vi "Scalar Bitpacked.vi"(8 "error in (no error)":errorcluster, 11 "Node Ptr":T1 format="%.0x") -> (0 "error out":errorcluster)   [LabVIEW 2020, in "FPGA Addon System Explorer.lvlib"]
uses:
  FPGA Addon System Explorer.lvlib
  <vilib>/NI VeriStand/Custom Device API/Custom Device API.lvlib
  Addon Shared/FPGA Addon Shared.lvlib
  Addon Shared/Types/FG Action.ctl
  Addon Shared/SubVIs/Constants.vi
  <vilib>/NI VeriStand/Custom Device API/Get Item Property (String).vi
  <vilib>/NI VeriStand/Custom Device API/Custom Device Item Ref.ctl
panel:
  out "Original Name":string
  in  "SHDocVw.IWebBrowser":refnum<k7>(container)
  in  "Reset":bool
  in  "Apply":bool
  in  "Number of Channels":u8
  in  "Header 2":cluster{"Section Name":string}={"Section Name"="Bitpacked Settings"}
  in  "Header":cluster{"Section Name":string}={"Section Name"="Section Settings"}
  in  "Description":string
  in  "Name":string
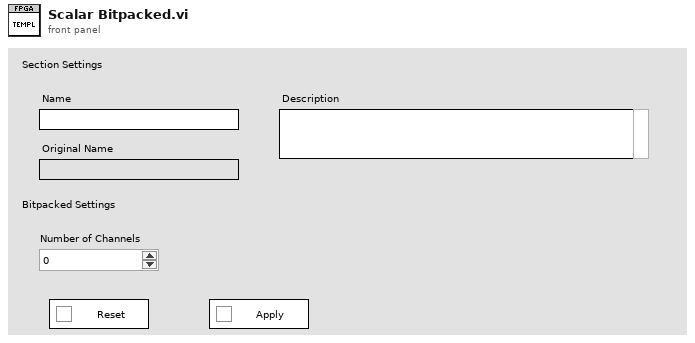
[diagram p1: front panel]
types:
  T1 = typedef "Custom Device API.lvlib/Custom Device Item Ref.ctl" = u64
  T2 = typedef "FPGA Addon Shared.lvlib/FG Action.ctl" = enum8{"GET", "SET"}
  T3 = typedef "FPGA Addon Shared.lvlib/Scalar Settings.ctl" = cluster{"Number of Channels":u8}
  T4 = typedef "FPGA Addon Shared.lvlib/Register Information.ctl" = cluster{"Name":string, "Data Type":T5, "Default Value":variant, "Attributes":variant}
  T5 = typedef "FPGA Addon Shared.lvlib/FPGA Addon Data Type.ctl" = enum8{"<Null>", "I8", "I16", "I32", "I64", "U8", "U16", "U32", "U64", "SGL", "Boolean", "Analog PWM In Settings", "Analog PWM In", "Digital PWM In Settings", "Digital PWM In", "Digital PWM Out", "Sine Out", "FXP", "FXP+/-24.5", "FXP+/-16.5", "FXP+/-32.8", "FXP+/-64.32", "FXP+/-16.7", "FXP+/-20.5", "FXP+/-27.5", "FXP+/-32.16", "FXP+16.3", "FXP+18.3", "Digital Static In", "Digital Static Out", "Digital Static In Settings", "Digital WSS Out", "Quad Encoder Settings", "Quad Encoder In", "Group"}
  T6 = typedef "Custom Device API.lvlib/Custom Device Item Info.ctl" = cluster{"Name":string, "Is Channel":bool, "GUID":string, "Is Waveform":bool}
  T7 = typedef "Custom Device API.lvlib/Custom Device Commands.ctl" = enum16{"Default", "Item renamed", "Shutdown", "Dynamic button pressed"}
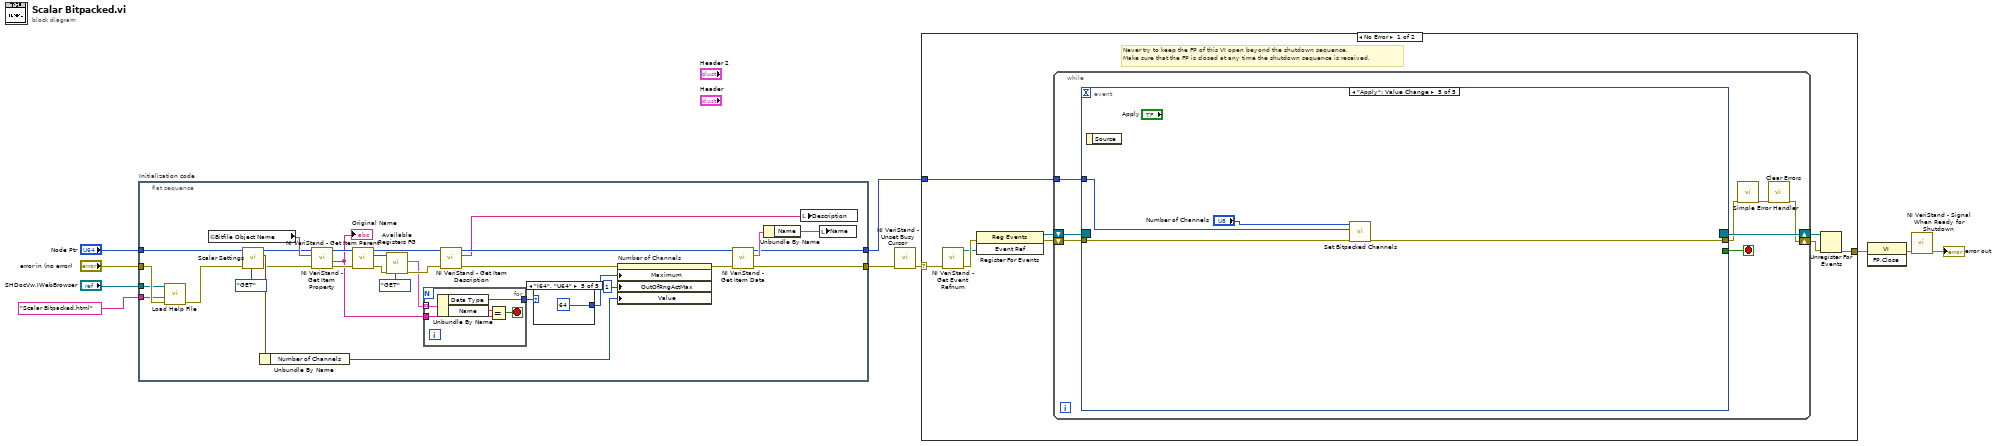
[diagram p0: block diagram]
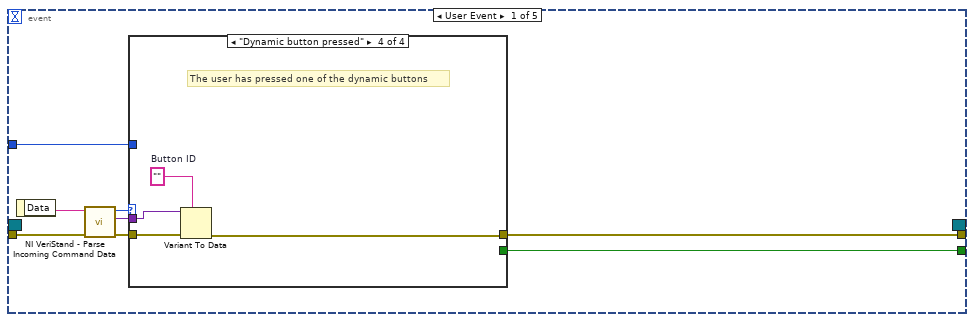
[diagram p2: hidden frame]
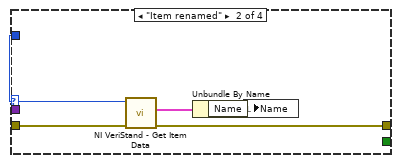
[diagram p4: hidden frame]
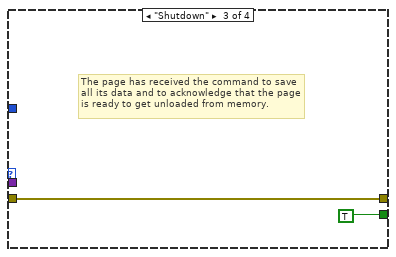
[diagram p5: hidden frame]
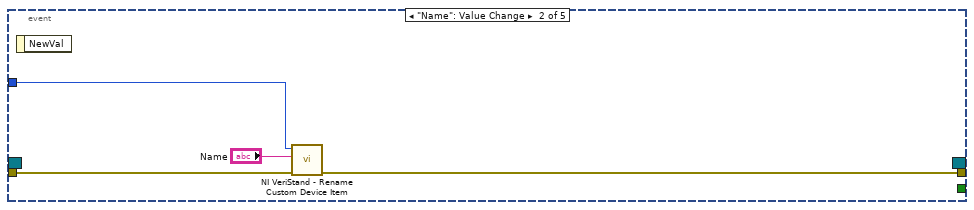
[diagram p6: hidden frame]
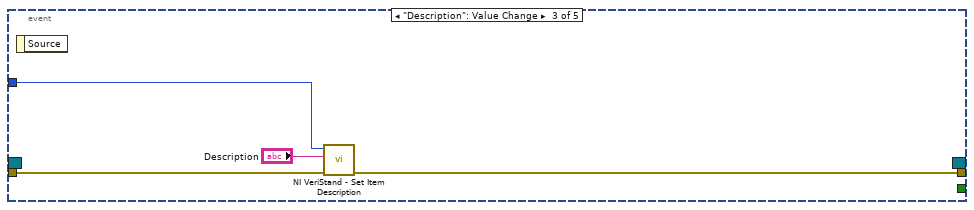
[diagram p7: hidden frame]
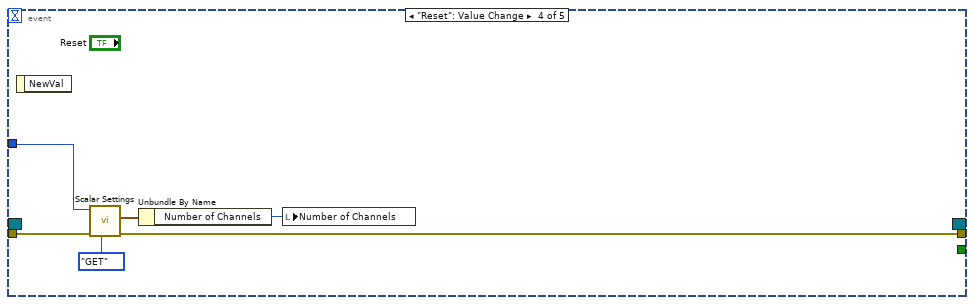
[diagram p8: hidden frame]
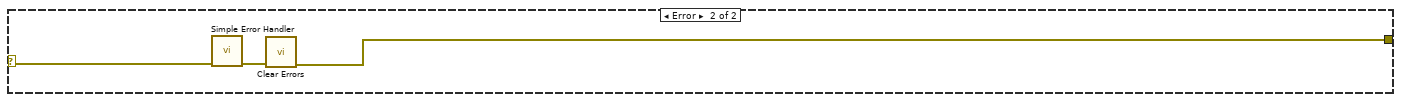
[diagram p9: hidden frame]
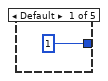
[diagram p10: hidden frame]
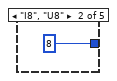
[diagram p11: hidden frame]
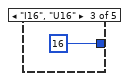
[diagram p12: hidden frame]
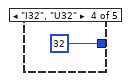
[diagram p13: hidden frame]
diagram:
  n1 = flat-sequence "Initialization code" {
    tunnel: "error in (no error)" -> [w15]
    tunnel: "Node Ptr" -> [w23]
    tunnel: [w37] -> w7
    tunnel: [w38] -> w5
    tunnel: "SHDocVw.IWebBrowser" -> [w13]
    tunnel: "Scalar Bitpacked.html" ("HTML File") -> [w12]
    frame #0 {
      n2 = call "Load Help File.vi"("error in (no error)"=w15, "HTML File to Load"=w12, "SHDocVw.IWebBrowser2"=w13) -> ("error out"=w14:errorcluster)  [unwired: 8 in]
      n3 = global read "Constants.vi" "Bitfile Object Name"() -> (w28:string)
      n4 = call "Scalar Settings.vi"("Action"=FG_Action."GET", "error in (no error)"=w14, "Item Ref"=w23) -> ("error out"=w22:errorcluster, "Scalar Settings"=w35:T3, "Item Ref out"=w21:T1)  [unwired: 6 in]
      n5 = Unbundle By Name(w35) -> ("Number of Channels"=w26:u8)
      n6 = call-poly <vilib>:"NI VeriStand - Get Item Property.vi"("error in (no error)"=w22, "Property Name"=w28, "Item Ref in"=w21) -> ("error out"=w19:errorcluster, "Value"=w11:string, "Item Ref out"=w20:T1)  [unwired: 5 in, 1 out]
      "Original Name" <- w11
      n7 = call <vilib>:"NI VeriStand - Get Item Parent.vi"("error in (no error)"=w19, "Item Ref in"=w20) -> ("error out"=w32:errorcluster, "Parent Ref"=w33:T1, "Item Ref out"=w34:T1)  [unwired: 6 in, 1 out]
      n8 = call "Available Registers FG.vi"("Action"=FG_Action."GET", "error in (no error)"=w32, "Item Ref"=w33) -> ("error out"=w31:errorcluster, "Available Registers"=w29:T4[])  [unwired: 6 in, 1 out]
      n9 = for {
        tunnel: w29 -> [w51] mode=indexing
        tunnel: w11 -> [w49]
        tunnel: [w47] -> w25
        stop <- w48 stop-if-true
        n10 = Unbundle By Name(w51) -> ("Data Type"=w47:T5, "Name"=w50:string)
        n11 = Equal?(x=w50, y=w49) -> (x = y?=w48:bool)
      }
      n12 = call <vilib>:"NI VeriStand - Get Item Description.vi"("error in (no error)"=w31, "Item Ref in"=w34) -> ("error out"=w18:errorcluster, "Description"=w40:string, "Item Ref out"=w41:T1)  [unwired: 7 out]
      n13 = case shown="\"I64\", \"U64\"" w25 {
        tunnel: [1 8 16 32 64] -> w24
        frame Default {
        }
        frame "I8", "U8" {
        }
        frame "I16", "U16" {
        }
        frame "I32", "U32" {
        }
        frame "I64", "U64" {
        }
      }
      n14 = property on="Number of Channels" class="DigNum (strict)"(error in=w18, "Maximum"=w24, "OutOfRngActMax"=u8 1 ("Response to Value Outside Limits:Maximum"), "Value"=w26) -> (error out=w17:errorcluster)  [unwired: 1 in, 1 out]
      n15 = call <vilib>:"NI VeriStand - Get Item Data.vi"("error in (no error)"=w17, "Item Ref in"=w41) -> ("error out"=w37:errorcluster, "Item Info"=w39:T6, "Item Ref out"=w38:T1)  [unwired: 7 out]
      n16 = Unbundle By Name(w39) -> ("Name"=w16:string)
      n17 = local write "Description"(w40) -> ()
      n18 = local write "Name"(w16) -> ()
    }
  }
  n19 = call <vilib>:"NI VeriStand - Unset Busy Cursor.vi"("error in (no error)"=w7) -> ("error out"=w6:errorcluster)  [unwired: 10 out]
  n20 = case shown="No Error" w6 {
    selector: w6 -> [w52 w109]
    tunnel: [w57 w107] -> w10
    tunnel: w5 -> [w53 _]
    frame No Error {
      # "Never try to keep the FP of this VI open beyond the shutdown sequence.\nMake sure that the FP is closed at any time the shutdown sequence is received."
      n21 = call <vilib>:"NI VeriStand - Get Event Refnum.vi"("error in (no error)"=w52) -> ("error out"=w60:errorcluster, "Event Ref"=w56:refnum<user-event>)  [unwired: 9 out]
      n22 = register-events(error in=w60, w56) -> (reference out=w54:refnum<event-registration>, error out=w55:errorcluster)  [unwired: 1 in]
      n23 = while {
        tunnel: w53 -> [w64]
        shift-right: [w61] -> w58
        shift-left: w55 -> [w67]
        shift-right: [w68] -> w59
        shift-left: w54 -> [w66]
        stop <- w65 stop-if-true
        n24 = event shown="[4] \"Apply\": Value Change" {
          selector: w66 -> [_ _ _ _ _]
          dyn-events: [_ _ _ _ _] -> w68
          timeout: _ -> [_ _ _ _ _]
          tunnel: w67 -> [w76 w92 w95 w102 w104]
          tunnel: [w72 _ _ _ _] -> w65
          tunnel: [w71 w91 w94 w98 w103] -> w63
          tunnel: w64 -> [w70 w90 w96 w100 w105]
          event User Event {
            n25 = event-data() -> ("Data"=w75:string)  [unwired: 1 out]
            n26 = call <vilib>:"NI VeriStand - Parse Incoming Command Data.vi"("error in (no error)"=w76, "Incoming data"=w75) -> ("error out"=w74:errorcluster, "Outgoing data"=w69:variant, "Action"=w73:T7)  [unwired: 7 out]
            n27 = case shown="\"Dynamic button pressed\"" w73 {
              tunnel: w74 -> [w77 w82 w83 w88]
              tunnel: [_ _ TRUE _] -> w72
              tunnel: [w77 w79 w83 w85] -> w71
              tunnel: w70 -> [_ w81 _ _]
              tunnel: w69 -> [_ _ _ w87]
              frame "Default", Default {
              }
              frame "Item renamed" {
                n28 = call <vilib>:"NI VeriStand - Get Item Data.vi"("error in (no error)"=w82, "Item Ref in"=w81) -> ("error out"=w79:errorcluster, "Item Info"=w80:T6)  [unwired: 8 out]
                n29 = Unbundle By Name(w80) -> ("Name"=w78:string)
                n30 = local write "Name"(w78) -> ()
              }
              frame "Shutdown" {
                # "The page has received the command to save all its data and to acknowledge that the page is ready to get unloaded from memory."
              }
              frame "Dynamic button pressed" {
                w86 = ""  # Button ID
                # "The user has pressed one of the dynamic buttons"
                n31 = Variant To Data(error in=w88, type=w86, Variant=w87) -> (error out=w85:errorcluster)  [unwired: 1 out]
              }
            }
          }
          event "Name": Value Change {
            n32 = event-data() -> ()  [unwired: 2 out]
            n33 = call <vilib>:"NI VeriStand - Rename Custom Device Item.vi"("error in (no error)"=w92, "New Name"="Name", "Item Ref in"=w90) -> ("error out"=w91:errorcluster)  [unwired: 1 in, 7 out]
          }
          event "Description": Value Change {
            n34 = event-data() -> ()  [unwired: 2 out]
            n35 = call <vilib>:"NI VeriStand - Set Item Description.vi"("error in (no error)"=w95, "Description"="Description", "Item Ref in"=w96) -> ("error out"=w94:errorcluster)  [unwired: 8 out]
          }
          event "Reset": Value Change {
            n36 = event-data() -> ()  [unwired: 2 out]
            n37 = call "Scalar Settings.vi"("Action"=FG_Action."GET", "error in (no error)"=w102, "Item Ref"=w100) -> ("error out"=w98:errorcluster, "Scalar Settings"=w99:T3)  [unwired: 6 in, 1 out]
            n38 = Unbundle By Name(w99) -> ("Number of Channels"=w97:u8)
            n39 = local write "Number of Channels"(w97) -> ()
          }
          event "Apply": Value Change {
            n40 = event-data() -> ()  [unwired: 2 out]
            n41 = call "Set Bitpacked Channels.vi"("error in (no error)"=w104, "Item Ref in"=w105, "Number of Channels"="Number of Channels") -> ("error out"=w103:errorcluster)  [unwired: 8 in]
          }
        }
        n42 = call <vilib>:"Simple Error Handler.vi"("error in (no error)"=w63) -> ("error out"=w62:errorcluster)  [unwired: 1 in, 7 out]
        n43 = call <vilib>:"Clear Errors.vi"("error in (no error)"=w62) -> ("error out"=w61:errorcluster)  [unwired: 1 in, 5 out]
      }
      n44 = Unregister For Events(event registration refnum=w59, error in=w58) -> (error out=w57:errorcluster)
    }
    frame Error {
      n45 = call <vilib>:"Simple Error Handler.vi"("error in (no error)"=w109) -> ("error out"=w108:errorcluster)  [unwired: 1 in, 7 out]
      n46 = call <vilib>:"Clear Errors.vi"("error in (no error)"=w108) -> ("error out"=w107:errorcluster)  [unwired: 1 in, 5 out]
    }
  }
  n47 = invoke class="VI" method="FP.Close"(error in=w10) -> (error out=w9:errorcluster)  [unwired: 2 in, 2 out]
  n48 = call <vilib>:"NI VeriStand - Signal When Ready for Shutdown.vi"("error in (no error)"=w9) -> ("error out"=→"error out":errorcluster)  [unwired: 10 out]
